vi "FeedDB.vi"(10 "feed GUID":string, 11 "Enum":T1) -> (3 "updated feeds (GUIDs)":string[](array[string]))   [LabVIEW 2023, in "GettingStartedWindow.lvlib" / "Feed_link.lvclass"]
uses:
  <resource>/modes/FRC/GSW/Classes/Feed_link/Feed_link.lvclass
  <resource>/modes/FRC/GSW/Classes/Feed_link/FeedDB_operation.ctl
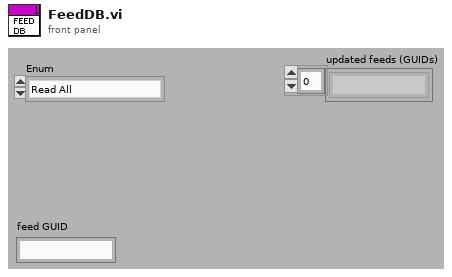
[diagram p1: front panel]
types:
  T1 = typedef "GettingStartedWindow.lvlib/Feed_link.lvclass/FeedDB_operation.ctl" = enum16{"Read All", "Append GUID"}
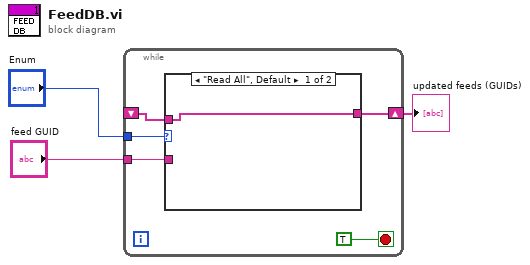
[diagram p0: block diagram]
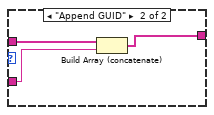
[diagram p2: hidden frame]
diagram:
  n1 = while {
    shift-right: [w4] -> w1
    shift-left: _ -> [w6]
    tunnel: "Enum" -> [w7]
    tunnel: "feed GUID" -> [w5]
    stop <- TRUE stop-if-true
    n2 = case shown="\"Read All\", Default" w7 {
      tunnel: w6 -> [w9 w12]
      tunnel: w5 -> [_ w11]
      tunnel: [w9 w10] -> w4
      frame "Read All", Default {
      }
      frame "Append GUID" {
        n3 = Build Array (concatenate)(w12, w11) -> (w10:string[])
      }
    }
  }
  "updated feeds (GUIDs)" <- w1
